vi "PLC_Frame.vi"(11 "Payload":string) -> (3 "Frame":string)   [LabVIEW 2018]
doc: "Use this template to build a VI to use as a subVI."
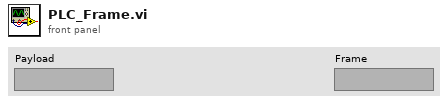
[diagram p1: front panel]
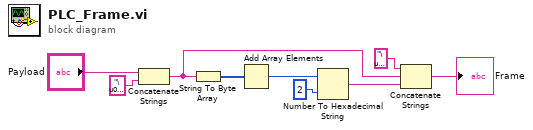
[diagram p0: block diagram]
diagram:
  n1 = Concatenate Strings("Payload", "\u0003") -> (w7:string)
  n2 = String To Byte Array(string=w7) -> (unsigned byte array=w6:u8[])
  n3 = Add Array Elements(numeric array=w6) -> (sum=w5:u8)
  n4 = Number To Hexadecimal String(1:i16 2 ("width (-)"), 2:w5) -> (0:w2:string)
  n5 = Concatenate Strings("\u0002", w7, w2) -> (→"Frame":string)
